vi "wiringPiSPIxSetupMode.vi"(8 "error in (no error)":errorcluster, 9 "Mode":T1, 10 "Speed":i32=4000000, 11 "SPI Device":T2) -> (0 "error out":errorcluster, 2 "return":i32, 3 "SPI Device out":T2)   [LabVIEW 2020, in "wiringPi.lvlib"]
doc: "<b>_______________________________________________________________</b>\n** Author: Juan José Villacorta\n** LabVIEW wrapper for C library <b> wiringPi </b>,\n** https://github.com/WiringPi/WiringPi\n<b>_______________________________________________________________</b>\n\n/*\n * wiringPiSPISetupMode:\n * Open the SPI device, and set it up, with the mode, etc.\n *********************************************************************************\n* number: SPI number (typically 0, on Compute Module 0-7).\n* channel: SPI channel (typically 0 or 1, on Compute Module 0-3).\n* speed: SPI clock speed in Hz (500,000 to 32,000,000).\n* mode: SPI mode (www.kernel.org/doc/Documentation/spi/spidev).\n* Return Value: File handle to the SPI bus, or -1 on error.\n */"
uses:
  wiringPi.lvlib
  Type Defs/SPI Dev.ctl
  Type Defs/SPI Channel.ctl
  Type Defs/SPI Device.ctl
  Type Defs/SPI Mode.ctl
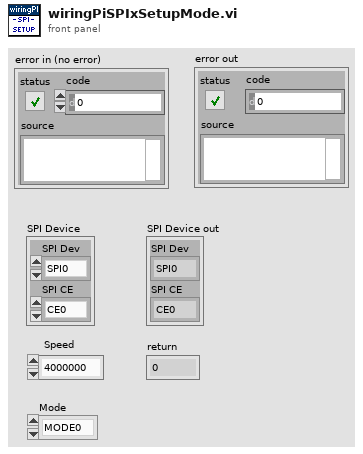
[diagram p1: front panel]
types:
  T1 = typedef "wiringPi.lvlib/SPI Mode.ctl" = enum32{"MODE0", "MODE1", "MODE2", "MODE3"}
  T2 = typedef "wiringPi.lvlib/SPI Device.ctl" = cluster{"SPI Dev":T3, "SPI CE":T4}
  T3 = typedef "wiringPi.lvlib/SPI Dev.ctl" = enum32{"SPI0", "SPI1"}
  T4 = typedef "wiringPi.lvlib/SPI Channel.ctl" = enum32{"CE0", "CE1", "CE2"}
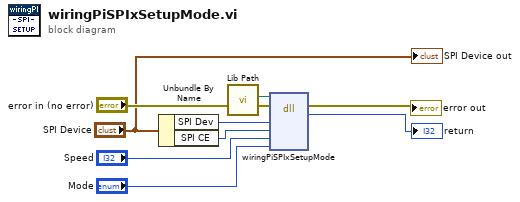
[diagram p0: block diagram]
diagram:
  n1 = Unbundle By Name("SPI Device") -> ("SPI Dev"=w5:T3, "SPI CE"=w4:T4)
  n2 = call "Lib Path.vi"() -> ("path out"=w1:path)  [unwired: 11 in]
  n3 = dll-call lib="libLVwiringPI.so" fn="wiringPiSPIxSetupMode"(path in=w1, error in="error in (no error)", "number"=w5, "channel"=w4, "speed"="Speed", "mode"="Mode") -> (error out=→"error out":errorcluster, "return type"=→"return":i32)  [unwired: 5 in, 1 out]
  "SPI Device out" <- "SPI Device"
